vi "PicoScope2000AWG.vi"(9 "Waveform Settings":T1 {"Start Frequency" min=1 max=1000000; "Wave Type" items=["Sine", "Square", "Triangle", "Ramp Up", "Ramp Down", "DC", "Arbitrary"]; "Sweep Type" items=["Up", "Down", "Up-Down", "Down-Up"]}, 10 "Handle In":i16, 11 "error in":errorcluster) -> (1 "Arbitrary\nWaveform Graph":u8[](graph), 2 "Handle Out":i16, 3 "error out":errorcluster)   [LabVIEW 2009]
doc: "This VI can be used to control the arbitrary waveform generator. Standard waveforms can be selected or arbitrary waveform can be selected under 'Wave Type'. There are three settings clusters: general settings that apply to both arbitrary and standard waveforms, settings that apply only to standard waveforms and settings that apply only to arbitrary waveforms. It is not necessary to connect all of these clusters if only using arbitrary waveforms or only using standard waveforms are required.\n\nWhen selecting arbitrary waveform, it is necessary to specify a text file containing the wave form. This text file should have a single value on each line in the range -1 to 1. For further information on the settings, see descriptions of ps3000aSetSigGenBuiltIn and ps3000aSetSigGenArbitrary."
uses:
  ps2000.dll
panel:
  out "Set Sig Gen Status":i16
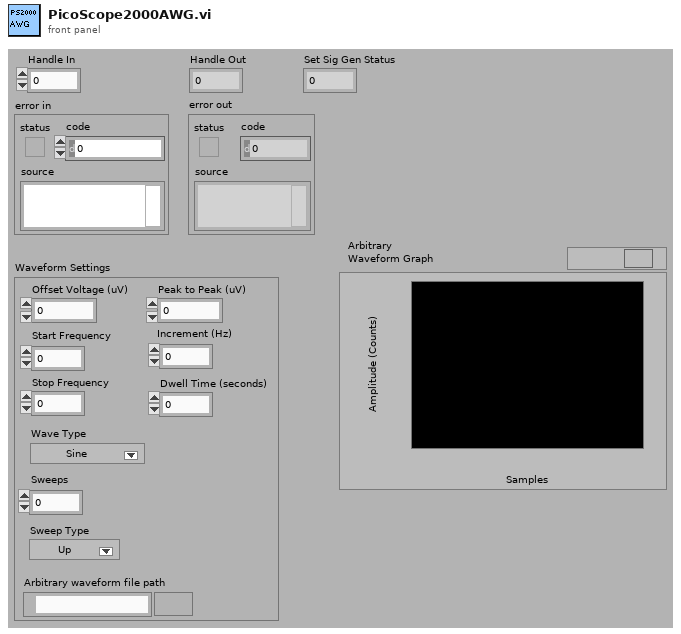
[diagram p1: front panel]
types:
  T1 = cluster{"Arbirary waveform file path":path, "Sweep Type":u32, "Sweeps":u32, "Wave Type":u32, "Start Frequency":sgl, "Stop Frequency":sgl, "Increment (Hz)":sgl, "Dwell Time (seconds)":sgl, "Offset Voltage (uV)":i32, "Peak to Peak (uV)":u32}
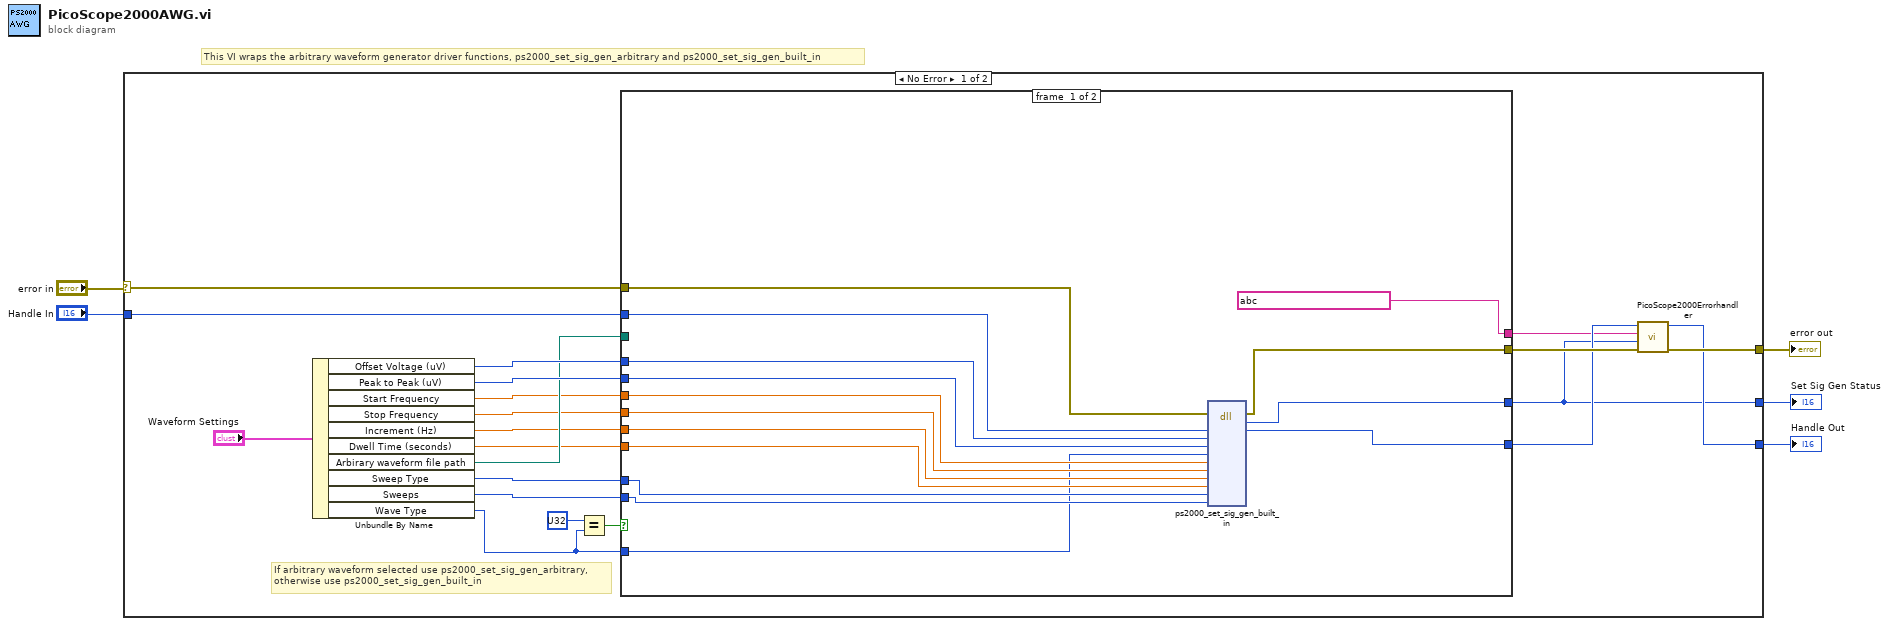
[diagram p0: block diagram]
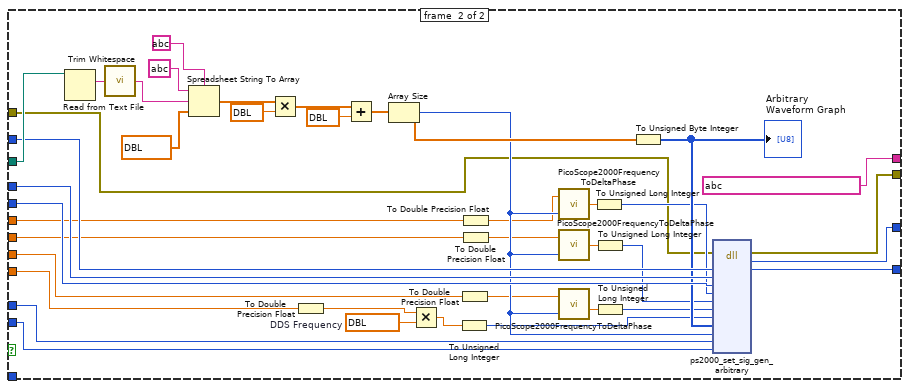
[diagram p2: hidden frame]
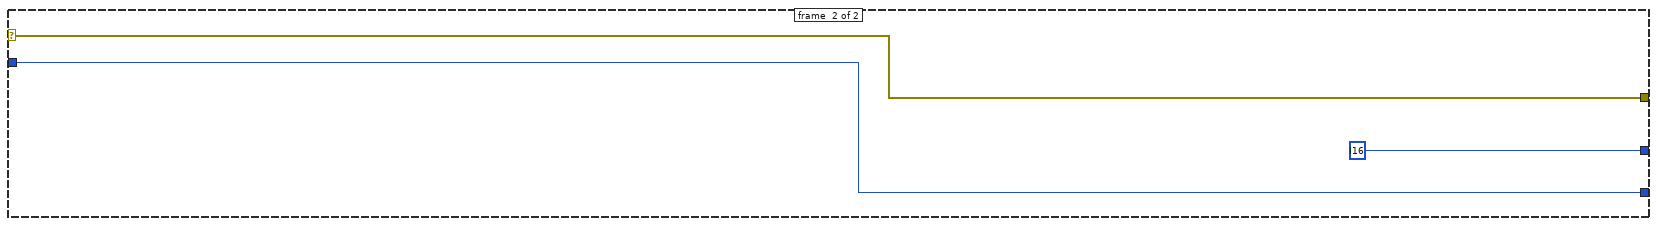
[diagram p3: hidden frame]
diagram:
  # "This VI wraps the arbitrary waveform generator driver functions, ps2000_set_sig_gen_arbitrary and ps2000_set_sig_gen_built_in"
  n1 = case shown="No Error" "error in" {
    selector: "error in" -> [w24 w84]
    tunnel: [w8 w83] -> w5
    tunnel: "Handle In" -> [w18 w83]
    tunnel: [w10 w84] -> w3
    tunnel: [w7 i16 ?] -> w1
    frame #0 {
      # "If arbitrary waveform selected use ps2000_set_sig_gen_arbitrary, \notherwise use ps2000_set_sig_gen_built_in"
      n2 = Unbundle By Name("Waveform Settings") -> ("Offset Voltage (uV)"=w22:i32, "Peak to Peak (uV)"=w21:u32, "Start Frequency"=w16:sgl, "Stop Frequency"=w15:sgl, "Increment (Hz)"=w14:sgl, "Dwell Time (seconds)"=w13:sgl, "Arbirary waveform file path"=w19:path, "Sweep Type"=w17:u32, "Sweeps"=w20:u32, "Wave Type"=w12:u32)
      n3 = Equal?(x=u32 ?, y=w12) -> (x = y?=w26:bool)
      n4 = case shown="True" w26 {
        tunnel: [w41 w72] -> w9
        tunnel: [w38 w81] -> w11
        tunnel: w20 -> [w37 w68]
        tunnel: w24 -> [w40 w45]
        tunnel: [w39 w71] -> w7
        tunnel: w22 -> [w30 w70]
        tunnel: w21 -> [w31 w69]
        tunnel: w19 -> [_ w67]
        tunnel: w18 -> [w29 w66]
        tunnel: w17 -> [w36 w65]
        tunnel: w16 -> [w32 w60]
        tunnel: w15 -> [w33 w59]
        tunnel: w14 -> [w34 w58]
        tunnel: w13 -> [w35 w49]
        tunnel: w12 -> [w28 _]
        tunnel: [string ? ("API function") string ? ("API function")] -> w6
        frame #0 {
          n5 = dll-call lib="ps2000.dll" fn="ps2000_set_sig_gen_built_in" ("ps3000.dll:_ps3000_open_unit@0")(error in=w40, "handle"=w29, "offsetVoltage"=w30, "pkToPk"=w31, "waveType"=w28, "startFrequency"=w32, "stopFrequency"=w33, "increment"=w34, "dwellTime"=w35, "sweepType"=w36, "sweeps"=w37) -> (error out=w38:errorcluster, "status"=w39:i16, "handle"=w41:i16)  [unwired: 11 in, 1 out]
        }
        frame #1 {
          w50 = dbl ?  # DDS Frequency
          n6 = Read from Text File(file (use dialog)=w67) -> (text=w44:string)  [unwired: 3 in, 3 out]
          n7 = call <vilib>:"Trim Whitespace.vi"("string"=w44) -> ("trimmed string"=w43:string)  [unwired: 1 in]
          n8 = Spreadsheet String To Array(delimiter (Tab)=string ?, format string=string ?, spreadsheet string=w43, array type (2D Dbl)=dbl[] ?) -> (array=w74:dbl[])
          n9 = Multiply(x=w74, y=dbl ? ("deltaPhaseIncrement")) -> (x*y=w76:dbl[])
          n10 = To Double Precision Float(number=w49) -> (double precision float=w48:dbl)
          n11 = Add(x=w76, y=dbl ? ("deltaPhaseIncrement")) -> (x+y=w73:dbl[])
          n12 = Array Size(array=w73) -> (size(s)=w54:i32)
          n13 = Multiply(x=w48, y=w50) -> (x*y=w47:dbl)
          n14 = To Unsigned Long Integer(number=w47) -> (unsigned 32bit integer=w46:u32)
          n15 = To Double Precision Float(number=w58) -> (double precision float=w51:dbl)
          n16 = To Double Precision Float(number=w60) -> (double precision float=w53:dbl)
          n17 = To Double Precision Float(number=w59) -> (double precision float=w52:dbl)
          n18 = call "PicoScope2000FrequencyToDeltaPhase.vi"("size"=w54, "frequency"=w53) -> ("deltaPhase"=w63:dbl)  [unwired: 1 in]
          n19 = call "PicoScope2000FrequencyToDeltaPhase.vi"("size"=w54, "frequency"=w52) -> ("deltaPhase"=w62:dbl)  [unwired: 1 in]
          n20 = call "PicoScope2000FrequencyToDeltaPhase.vi"("size"=w54, "frequency"=w51) -> ("deltaPhase"=w61:dbl)  [unwired: 1 in]
          n21 = To Unsigned Long Integer(number=w63) -> (unsigned 32bit integer=w57:u32)
          n22 = To Unsigned Long Integer(number=w62) -> (unsigned 32bit integer=w56:u32)
          n23 = To Unsigned Long Integer(number=w61) -> (unsigned 32bit integer=w55:u32)
          n24 = To Unsigned Byte Integer(number=w73) -> (unsigned 8bit integer=w64:u8[])
          "Arbitrary\nWaveform Graph" <- w64
          n25 = dll-call lib="PS2000.dll" fn="ps2000_set_sig_gen_arbitrary"(error in=w45, "handle"=w66, "offsetvoltage"=w70, "pktopk"=w69, "startDeltaPhase"=w57, "stopDeltaPhase"=w56, "deltaPhaseIncrement"=w55, "dwellCount"=w46, "arbitraryWaveform"=w64, "arbitraryWaveformSize"=w54, "sweepType"=w65, "sweeps"=w68) -> (error out=w81:errorcluster, "return"=w71:i16, "handle"=w72:i16)  [unwired: 12 in, 1 out]
        }
      }
      n26 = call "PicoScope2000Errorhandler.vi"("Handle in"=w9, "API function"=w6, "Return"=w7, "error in (no error)"=w11) -> ("Handle out"=w8:i16, "error out"=w10:errorcluster)  [unwired: 5 in]
    }
    frame #1 {
    }
  }
  "Handle Out" <- w5
  "error out" <- w3
  "Set Sig Gen Status" <- w1
